vi "user32 PrintWindow.vi"(0 "hwnd":u64, 5 "hdcBlt":u64, 7 "nFlags":u32=2, 11 "error in":errorcluster) -> (4 "return value":i32, 15 "error out":errorcluster)   [LabVIEW 2020, in "RemoteVI.lvlib"]
doc: "Asks the window hwnd to draw itself into the device context hdcBlt through user32.dll PrintWindow (stdcall, called in any thread). With nFlags 2 PW_RENDERFULLCONTENT the window's own content is captured whether or not it is visible, covered or on another monitor - also a layered window with alpha 0. hdcBlt is normally a memory DC with a bitmap of the window's size selected into it. return value is the Win32 BOOL: non-zero on success, 0 on failure. When error in carries an error the DLL is not called. Generated by scripts\\Build Win32 Wrappers.vi - do not edit by hand, rebuild it."
uses:
  RemoteVI.lvlib
  user32.dll
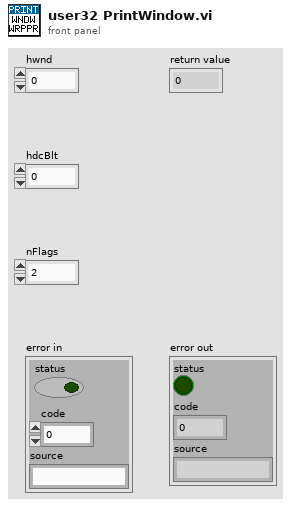
[diagram p1: front panel]
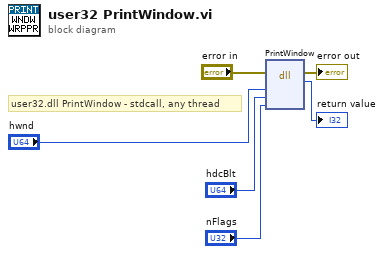
[diagram p0: block diagram]
diagram:
  # "user32.dll PrintWindow - stdcall, any thread"
  n1 = dll-call lib="user32.dll" fn="PrintWindow"(error in="error in", "hwnd"="hwnd", "hdcBlt"="hdcBlt", "nFlags"="nFlags") -> (error out=→"error out":errorcluster, →"return value":i32)  [unwired: 5 in, 1 out]
